vi "user32 ChildWindowFromPointEx.vi"(0 "hwnd":u64, 5 "pt":u64, 7 "flags":u32=5, 11 "error in":errorcluster) -> (4 "child":u64, 15 "error out":errorcluster)   [LabVIEW 2020, in "RemoteVI.lvlib"]
doc: "Returns the child window of hwnd that contains a point through user32.dll ChildWindowFromPointEx (stdcall, called in any thread). The point is in hwnd's CLIENT coordinates and travels BY VALUE as a POINT {LONG x, LONG y}, passed here as one U64 pt with x in the low and y in the high 32 bits - the POINT's memory image, which is how an 8-byte struct is passed by value on x64 (one register) and on x86 (two stack slots). Only immediate children are searched; call it again with the answer for deeper ones. flags 5 (default) = CWP_SKIPINVISIBLE 1 + CWP_SKIPTRANSPARENT 4; 2 CWP_SKIPDISABLED. child is hwnd itself when no child contains the point and 0 when the point is outside hwnd. When error in carries an error the DLL is not called. Generated by scripts\\Build Win32 Wrappers.vi - do not edit by hand, rebuild it."
uses:
  RemoteVI.lvlib
  user32.dll
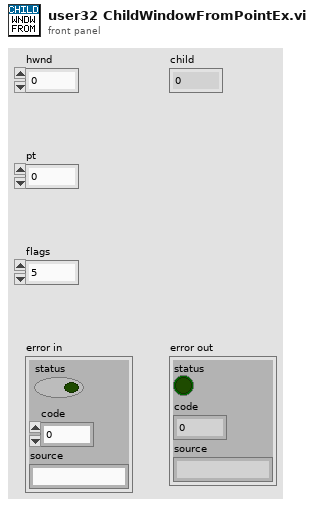
[diagram p1: front panel]
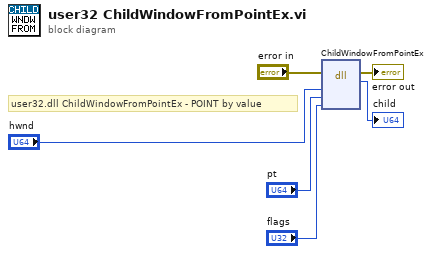
[diagram p0: block diagram]
diagram:
  # "user32.dll ChildWindowFromPointEx - POINT by value"
  n1 = dll-call lib="user32.dll" fn="ChildWindowFromPointEx"(error in="error in", "hwnd"="hwnd", "pt"="pt", "flags"="flags") -> (error out=→"error out":errorcluster, →"child":u64)  [unwired: 5 in, 1 out]
